vi "Get View VI Reference.vi"(8 "error in (no error)":errorcluster, 11 "View In":refnum<class "View.lvclass">) -> (0 "error out":errorcluster, 2 "View VI Reference":refnum<vi>, 3 "View Out":refnum<class "View.lvclass">)   [LabVIEW 2020, in "View.lvclass"]
doc: "Get the View VI referene as set by the Set View VI Reference.vi method."
uses:
  View.lvclass
  C:/git/astemes-triarc-framework/source/Framework/Process/Process.lvclass
  Process/Public/Lifecycle/Lifecycle State.ctl
  Process/Process.lvclass/Process.ctl
  View.lvclass/View.ctl
  Process/Protected/Messaging/Async Request Message.vi
  Process/Private/SubVIs/Handle Debug Data.vi
  Logging/Log Debug.vi
  <vilib>/AdvancedString/1D String Array to Delimited String.vi
  <vilib>/Utility/High Resolution Relative Seconds.vi
  Synchronous Request Callback/Synchronous Request Callback.lvclass
  C:/git/astemes-triarc-framework/source/Framework/Callback/Callback.lvclass
  Process/Process.lvclass
  C:/git/astemes-triarc-framework/source/Framework/Logging/Logging.lvclass
  <vilib>/Utility/error.llb/Error Cluster From Error Code.vi
  Synchronous Request Callback/Create.vi
  Process/Public/Read Name.vi
  Process/Private/SubVIs/Wait for Response Message.vi
  <vilib>/ErrorRing/Error Ring.xnode
  Callback/Callback.lvclass
  Logging/Logging.lvclass
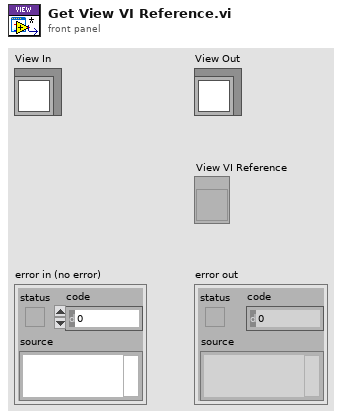
[diagram p1: front panel]
types:
  T1 = typedef "Process.lvclass/Lifecycle State.ctl" = enum16{"Uninitialized", "Initialized", "Started", "Running", "Stopped", "Finished"}
  T2 = typedef "Process.lvclass/API Mode.ctl" = enum16{"Send Message", "Handle Message"}
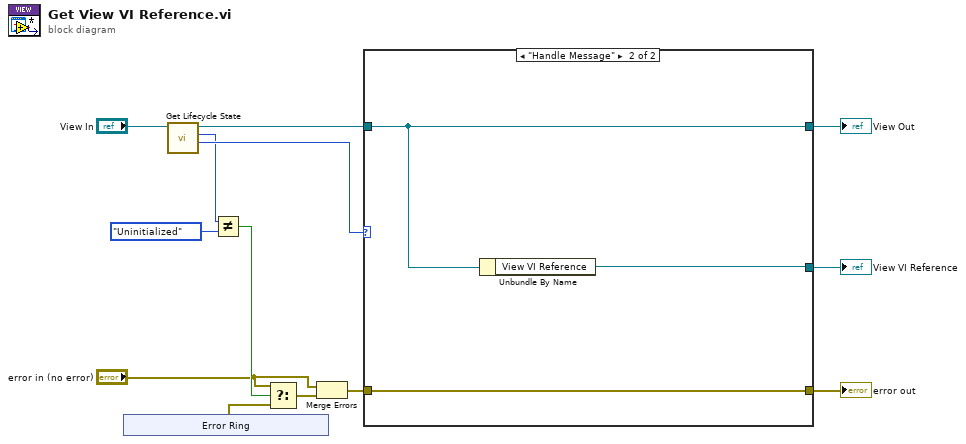
[diagram p0: block diagram]
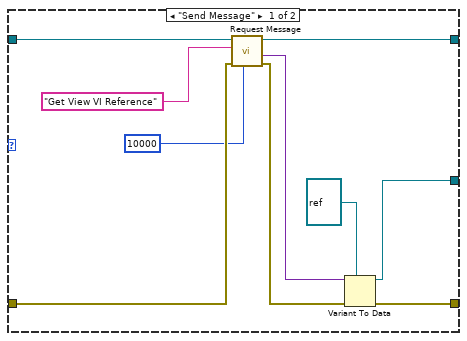
[diagram p2: hidden frame]
diagram:
  n1 = xnode "Error Ring"() -> ("error out"=w3:errorcluster)
  n2 = call "Get Lifecycle State.vi"("Process In"="View In") -> ("API Mode"=w8:T2, "Lifecycle State"=w6:T1, "Process Out"=w9:refnum<class "View.lvclass">)  [unwired: 7 in, 1 out]
  n3 = Not Equal?(x=w6, y=Lifecycle_State."Uninitialized") -> (x != y?=w4:bool)
  n4 = Select(t="error in (no error)", s=w4, f=w3) -> (s? t:f=w1:errorcluster)
  n5 = Merge Errors("error in (no error)", w1) -> (w7:errorcluster)
  n6 = case shown="\"Handle Message\"" w8 {
    tunnel: [w23 w25] -> w12
    tunnel: [w20 w24] -> w11
    tunnel: [w17 w26] -> w10
    tunnel: w9 -> [w16 w25]
    tunnel: w7 -> [w15 w24]
    frame "Send Message" {
      n7 = call "Request Message.vi"("timeout in ms (-1)"=10000, "error in (no error)"=w15, "Request Message"="Get View VI Reference", "Process In"=w16) -> ("error out"=w22:errorcluster, "Response Message Data"=w18:variant, "Process Out"=w23:refnum<class "View.lvclass">)  [unwired: 3 in, 2 out]
      n8 = Variant To Data(error in=w22, type=refnum<vi> refnum ("UI View VI Reference"), Variant=w18) -> (data=w17:refnum<vi>, error out=w20:errorcluster)
    }
    frame "Handle Message" {
      n9 = Unbundle By Name(w25) -> ("View VI Reference"=w26:refnum<vi>)
    }
  }
  "error out" <- w11
  "View Out" <- w12
  "View VI Reference" <- w10
